vi "Sim_Check_Safety.vi"(10 "Settings":T3={"UI Update Interval (ms)"=200, "Max dt (s)"=1.0, "Initial SOC (%)"=50.0, "Rest Voltage (V)"=12.0, "Ambient Temperature (degC)"=25.0, "Voltage Time Constant (s)"=5.0, "Current Time Constant (s)"=1.0, "Thermal Time Constant (s)"=120.0, "Heating Coefficient (degC/s per A^2)"=0.002, "SOC Speed Factor"=1.0, "Charge Complete SOC (%)"=100.0, "Discharge Complete SOC (%)"=0.0, "Max Voltage Limit (V)"=15.0, "Max Current Limit (A)"=10.0, "Max Temperature Limit (degC)"=45.0, "Max C-Rate (1/h)"=5.0, "Max Duration (min)"=600.0, "History Length (samples)"=3000, "Inject E-Stop"=FALSE, "Inject Overvoltage"=FALSE, "Inject Overcurrent"=FALSE, "Inject Overtemperature"=FALSE}, 11 "Sim Data in":T1) -> (2 "Fault Active?":bool, 3 "Sim Data out":T1)   [LabVIEW 2019]
doc: "Simulated safety check - NOT a substitute for a BMS or hardware interlock. Priority: 1 E-Stop injection, 2 overvoltage, 3 overcurrent, 4 overtemperature (each: injection OR value above the DEMO limit), 5 output interlock (supply and load both on). On a fault: Fault latched with code, reason and first fault time, both simulated outputs OFF, both half-cycle flags cleared. While a fault is ALREADY latched the Status Message is left as it is, so command messages (Start blocked, reset refused) stay visible. Without a fault the data passes through unchanged (a latched fault is cleared only by Reset Fault in the main VI)."
uses:
  Sim_Data.ctl
  Test_State_Enum2.ctl
  Sim_Settings.ctl
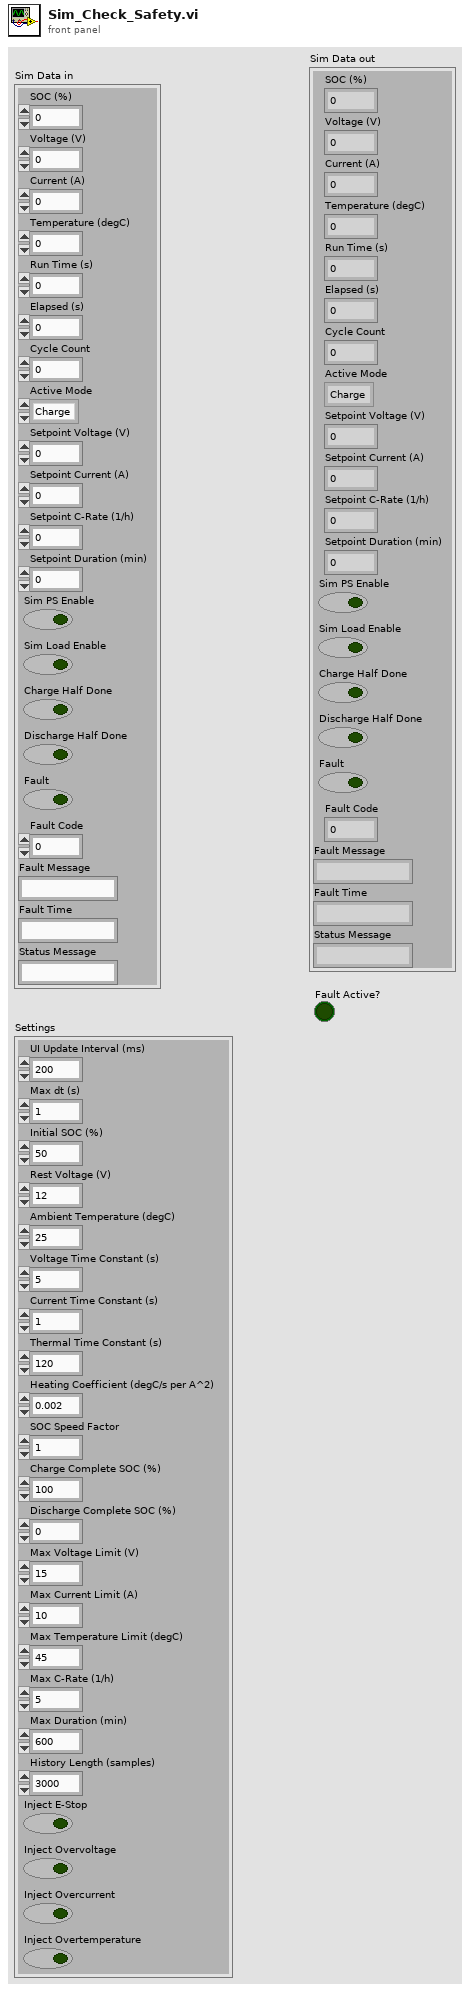
[diagram p1: front panel]
types:
  T1 = typedef "Sim_Data.ctl" = cluster{"SOC (%)":dbl, "Voltage (V)":dbl, "Current (A)":dbl, "Temperature (degC)":dbl, "Run Time (s)":dbl, "Elapsed (s)":dbl, "Cycle Count":u32, "Active Mode":T2, "Setpoint Voltage (V)":dbl, "Setpoint Current (A)":dbl, "Setpoint C-Rate (1/h)":dbl, "Setpoint Duration (min)":dbl, "Sim PS Enable":bool, "Sim Load Enable":bool, "Charge Half Done":bool, "Discharge Half Done":bool, "Fault":bool, "Fault Code":i32, "Fault Message":string, "Fault Time":string, "Status Message":string}
  T2 = typedef "Test_State_Enum2.ctl" = enum16{"Charge", "Discharge"}
  T3 = typedef "Sim_Settings.ctl" = cluster{"UI Update Interval (ms)":i32, "Max dt (s)":dbl, "Initial SOC (%)":dbl, "Rest Voltage (V)":dbl, "Ambient Temperature (degC)":dbl, "Voltage Time Constant (s)":dbl, "Current Time Constant (s)":dbl, "Thermal Time Constant (s)":dbl, "Heating Coefficient (degC/s per A^2)":dbl, "SOC Speed Factor":dbl, "Charge Complete SOC (%)":dbl, "Discharge Complete SOC (%)":dbl, "Max Voltage Limit (V)":dbl, "Max Current Limit (A)":dbl, "Max Temperature Limit (degC)":dbl, "Max C-Rate (1/h)":dbl, "Max Duration (min)":dbl, "History Length (samples)":i32, "Inject E-Stop":bool, "Inject Overvoltage":bool, "Inject Overcurrent":bool, "Inject Overtemperature":bool}
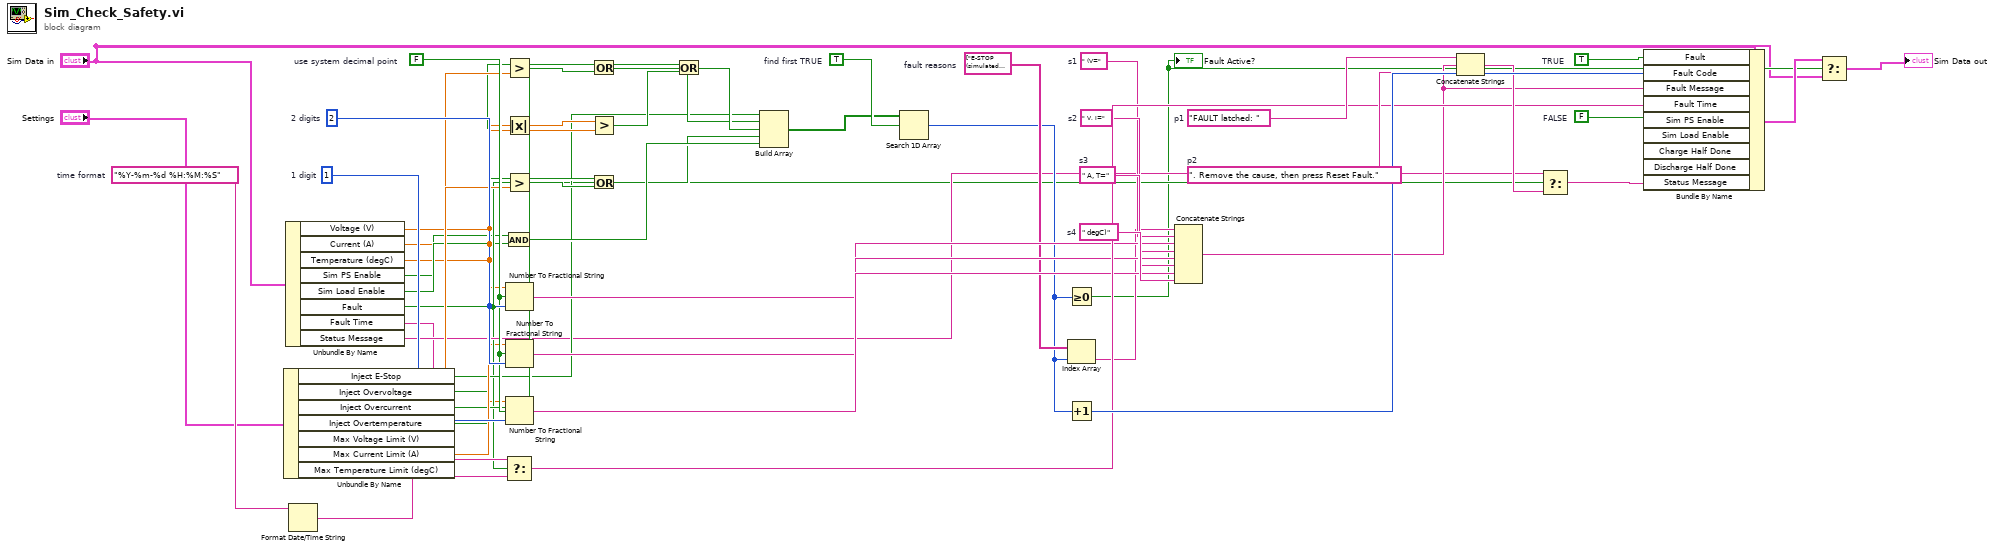
[diagram p0: block diagram]
diagram:
  w53 = FALSE  # FALSE
  w52 = TRUE  # TRUE
  w48 = ". Remove the cause, then press Reset Fault."  # p2
  w47 = "FAULT latched: "  # p1
  w44 = "%Y-%m-%d %H:%M:%S"  # time format
  w42 = " degC)"  # s4
  w41 = " A, T="  # s3
  w40 = " V, I="  # s2
  w39 = " (V="  # s1
  w35 = 1  # 1 digit
  w34 = 2  # 2 digits
  w33 = FALSE  # use system decimal point
  w31 = string[] ["E-STOP (simulated fault injection)", "OVERVOLTAGE (simulated - above demo Max Voltage Limit)", "OVERCURRENT (simulated - above demo Max Current Limit)", "OVERTEMPERATURE (simulated - above demo Max Temperature Limit)", "OUTPUT INTERLOCK (supply and load both enabled)"]  # fault reasons
  w29 = TRUE  # find first TRUE
  n1 = Unbundle By Name("Settings") -> ("Inject E-Stop"=w13:bool, "Inject Overvoltage"=w14:bool, "Inject Overcurrent"=w15:bool, "Inject Overtemperature"=w16:bool, "Max Voltage Limit (V)"=w17:dbl, "Max Current Limit (A)"=w18:dbl, "Max Temperature Limit (degC)"=w19:dbl)
  n2 = Unbundle By Name("Sim Data in") -> ("Voltage (V)"=w5:dbl, "Current (A)"=w6:dbl, "Temperature (degC)"=w7:dbl, "Sim PS Enable"=w8:bool, "Sim Load Enable"=w9:bool, "Fault"=w10:bool, "Fault Time"=w11:string, "Status Message"=w12:string)
  n3 = Format Date/Time String(time format string (%c)=w44) -> (date/time string=w45:string)  [unwired: 1 in, 1 out]
  n4 = Greater?(x=w5, y=w17) -> (0:w20:bool)
  n5 = Absolute Value(x=w6) -> (abs(x)=w22:dbl)
  n6 = Greater?(x=w7, y=w19) -> (0:w25:bool)
  n7 = And(x=w8, y=w9) -> (x .and. y?=w27:bool)
  n8 = Number To Fractional String(use system decimal point (T)=w33, number=w5, precision (6)=w34) -> (F-format string=w36:string)  [unwired: 1 out]
  n9 = Number To Fractional String(use system decimal point (T)=w33, number=w6, precision (6)=w34) -> (F-format string=w37:string)  [unwired: 1 out]
  n10 = Number To Fractional String(use system decimal point (T)=w33, number=w7, precision (6)=w35) -> (F-format string=w38:string)  [unwired: 1 out]
  n11 = Select(t=w11, s=w10, f=w45) -> (s? t:f=w46:string)
  n12 = Or(x=w14, y=w20) -> (x .or. y?=w21:bool)
  n13 = Greater?(x=w22, y=w18) -> (0:w23:bool)
  n14 = Or(x=w16, y=w25) -> (x .or. y?=w26:bool)
  n15 = Or(x=w15, y=w23) -> (x .or. y?=w24:bool)
  n16 = Build Array(w13, w21, w24, w26, w27) -> (w28:bool[])
  n17 = Search 1D Array(1D array=w28, element=w29) -> (index of element=w30:i32)  [unwired: 1 in]
  n18 = Greater Or Equal To 0?(x=w30) -> (x >= 0?=w4:bool)
  "Fault Active?" <- w4
  n19 = Index Array(array=w31, index=w30) -> (element=w32:string)
  n20 = Increment(x=w30) -> (x+1=w51:i32)
  n21 = Concatenate Strings(w32, w39, w36, w40, w37, w41, w38, w42) -> (w43:string)
  n22 = Concatenate Strings(w47, w43, w48) -> (w49:string)
  n23 = Select(t=w12, s=w10, f=w49) -> (s? t:f=w50:string)
  n24 = Bundle By Name(cluster="Sim Data in", "Fault"=w52, "Fault Code"=w51, "Fault Message"=w43, "Fault Time"=w46, "Sim PS Enable"=w53, "Sim Load Enable"=w53, "Charge Half Done"=w53, "Discharge Half Done"=w53, "Status Message"=w50) -> (w54:T1)
  n25 = Select(t=w54, s=w4, f="Sim Data in") -> (s? t:f=→"Sim Data out":T1)
